vi "kernel32 OpenProcess.vi"(0 "process ID":u32, 5 "dwDesiredAccess":u32=4096, 7 "bInheritHandle":i32, 11 "error in":errorcluster) -> (4 "HANDLE":u64, 15 "error out":errorcluster)   [LabVIEW 2020, in "RemoteVI.lvlib"]
doc: "Opens a handle to the process process ID through kernel32.dll OpenProcess (stdcall, called in any thread). RemoteVI asks only for PROCESS_QUERY_LIMITED_INFORMATION (0x1000), which is enough to read the program's path (kernel32 QueryFullProcessImageNameW.vi) and is granted for most processes of the same user. HANDLE is 0 on failure. Close it with kernel32 CloseHandle.vi. When error in carries an error the DLL is not called. Generated by scripts\\Build Win32 Wrappers.vi - do not edit by hand, rebuild it."
uses:
  RemoteVI.lvlib
  kernel32.dll
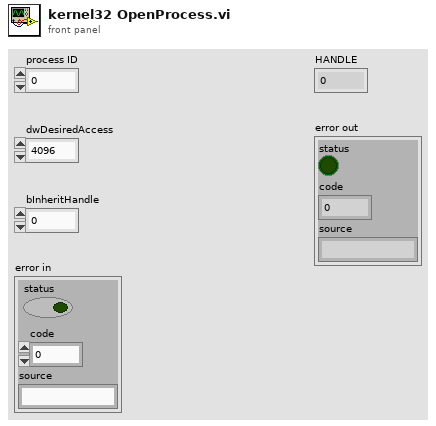
[diagram p1: front panel]
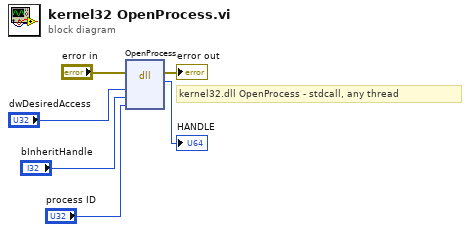
[diagram p0: block diagram]
diagram:
  # "kernel32.dll OpenProcess - stdcall, any thread"
  n1 = dll-call lib="kernel32.dll" fn="OpenProcess"(error in="error in", "dwDesiredAccess"="dwDesiredAccess", "bInheritHandle"="bInheritHandle", "dwProcessId"="process ID") -> (error out=→"error out":errorcluster, →"HANDLE":u64)  [unwired: 5 in, 1 out]
